vi "RemoteVI App Settings.vi"() -> ()   [LabVIEW 2020]
doc: "Screen Settings of RemoteVI Application Example.vi: settings of the station (simulated - nothing is stored). Save confirms in a LabVIEW dialog. Runs until the notifier RemoteVI Application Example fires (the main VI quits)."
panel:
  out "Status":string
  in  "Save":bool
  in  "Export Folder":path=path "C:/Data/Export"
  in  "Export Automatically":bool=TRUE
  in  "Keep Logs (days)":dbl=30.0
  in  "Sample Interval (ms)":dbl=100.0
  in  "Units":enum16{"SI (bar, degC)", "US (psi, degF)"}(ring)
  in  "Operator":string="Shift A"
  in  "Station Name":string="Cooling loop test bench"
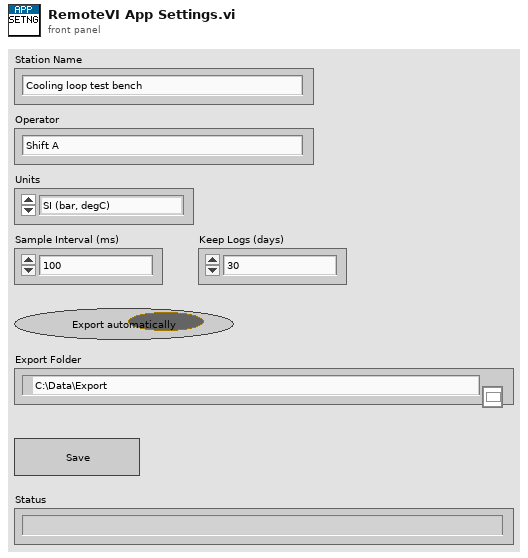
[diagram p1: front panel]
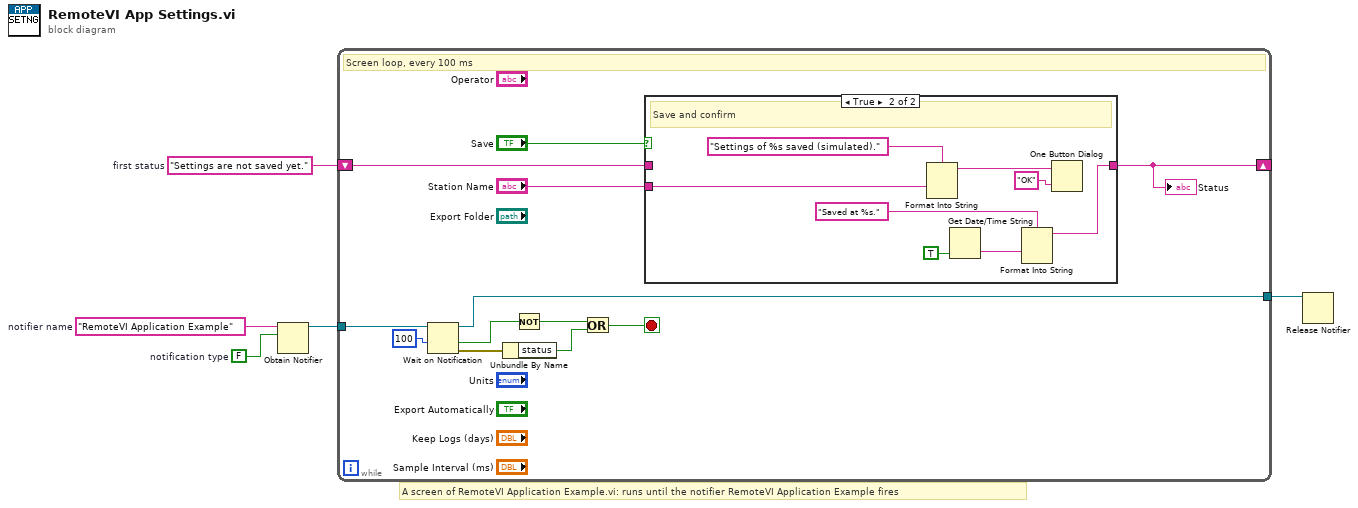
[diagram p0: block diagram]
diagram:
  w3 = FALSE  # notification type
  w2 = "RemoteVI Application Example"  # notifier name
  w1 = "Settings are not saved yet."  # first status
  # "A screen of RemoteVI Application Example.vi: runs until the notifier RemoteVI Application Example fires"
  n1 = Obtain Notifier(name (unnamed)=w2, notification data type=w3) -> (notifier out=w4:refnum<notifier>)  [unwired: 2 in, 2 out]
  n2 = while {
    shift-right: [w8] -> _
    shift-left: w1 -> [w7]
    tunnel: w4 -> [w6]
    tunnel: [w12] -> w5
    stop <- w17 stop-if-true
    # "Screen loop, every 100 ms"
    n3 = Wait on Notification(notifier=w6, timeout in ms (-1)=100) -> (notifier out=w12:refnum<notifier>, timed out?=w13:bool, error out=w14:errorcluster)  [unwired: 2 in, 1 out]
    n4 = Unbundle By Name(w14) -> ("status"=w16:bool)
    n5 = Not(x=w13) -> (.not. x?=w15:bool)
    n6 = Or(x=w15, y=w16) -> (x .or. y?=w17:bool)
    n7 = case shown="True" "Save" {
      tunnel: "Station Name" -> [_ w19]
      tunnel: w7 -> [w18 _]
      tunnel: [w18 w26] -> w8
      frame False {
        # "Not pressed"
      }
      frame True {
        # "Save and confirm"
        n8 = Format Into String(format string="Settings of %s saved (simulated).", w19) -> (resulting string=w21:string)  [unwired: 2 in, 1 out]
        n9 = Get Date/Time String(want seconds? (F)=TRUE) -> (time string=w24:string)  [unwired: 3 out]
        n10 = Format Into String(format string="Saved at %s.", w24) -> (resulting string=w26:string)  [unwired: 2 in, 1 out]
        n11 = One Button Dialog(message=w21, button name ("OK")="OK") -> ()  [unwired: 1 out]
      }
    }
    "Status" <- w8
  }
  n12 = Release Notifier(notifier=w5) -> ()  [unwired: 2 in, 3 out]
